vi "[ex ce] Levenberg Marquardt with independent parameter.vi"() -> ()   [LabVIEW 2021]
doc: "CE-Math example.\n\n::: CalcExpress Toolkit :::\nCopyright (c) 2000-2026 Konstantin Shifershteyn. All rights reserved."
uses:
  <vilib>/Analysis/2dsp.llb/1D Convolution (DBL).vi
  <vilib>/Analysis/NI_AALPro.lvlib
panel:
  out "error out":errorcluster
  in  "Initial Guess Coef.":cluster{"a":dbl, "b":dbl, "DC":dbl}={"a"=1.0, "b"=1.0, "DC"=0.0}
  out "Computed Coefficients":cluster{"a":dbl, "b":dbl, "DC":dbl}
  out "MSE":dbl
  in  "model description":T1={"model"="Conv( Sig , a*exp(-MesData/b)) + DC", "Parameters"=["a", "b", "DC"], "x-variable"="MesData"}
  in  "DC":dbl=4.0 caption="DC  =" format="%.1f"
  in  "Noise Amp.":dbl=2.0 caption="Noise Amplitude  =" format="%.1f"
  in  "dt, sec":dbl=0.5
  in  "a":dbl=3.0 caption="a ="
  in  "b":dbl=3.5 caption="b ="
  out "XY Graph":cluster{dbl[], dbl[]}[](graph)
  in  "Control Signal (Sig)":dbl[](array[slide])=[0.04081632653061224, 0.0510204081632653, 0.030612244897959183, 0.0510204081632653, 0.04081632653061224, 0.0510204081632653, 0.030612244897959183, 0.061224489795918366, 0.030612244897959183, 0.030612244897959183, 0.04081632653061224, 0.0510204081632653, 0.030612244897959183, 0.0510204081632653, 0.1020408163265306, 0.04081632653061224, 0.030612244897959183, 0.04081632653061224, 0.030612244897959183, 0.04081632653061224, 0.030612244897959183, 0.1020408163265306, 0.2346938775510204, 0.4387755102040816, 0.673469387755102, 0.7959183673469387, 0.9183673469387754, 0.8979591836734693, 0.8163265306122448, 0.7346938775510203, 0.6122448979591836, 0.4081632653061224, 0.24489795918367346, 0.11224489795918366, 0.061224489795918366, 0.07142857142857142, 0.07142857142857142, 0.030612244897959183, 0.0510204081632653, 0.061224489795918366, 0.07142857142857142, 0.04081632653061224, 0.030612244897959183, 0.0510204081632653, 0.0510204081632653, 0.04081632653061224, 0.030612244897959183, 0.030612244897959183, 0.061224489795918366, 0.02040816326530612, 0.030612244897959183, 0.061224489795918366, 0.030612244897959183, 0.0510204081632653, 0.030612244897959183, 0.030612244897959183, 0.02040816326530612, 0.030612244897959183, 0.04081632653061224, 0.030612244897959183, 0.04081632653061224, 0.09183673469387754, 0.2040816326530612, 0.32653061224489793, 0.4081632653061224, 0.36734693877551017, 0.25510204081632654, 0.13265306122448978, 0.061224489795918366, 0.030612244897959183, 0.030612244897959183, 0.061224489795918366, 0.0510204081632653, 0.0510204081632653, 0.0510204081632653, 0.04081632653061224, 0.04081632653061224, 0.030612244897959183, 0.02040816326530612, 0.030612244897959183, 0.030612244897959183, 0.01020408163265306, 0.0510204081632653, 0.0510204081632653, 0.030612244897959183, 0.030612244897959183, 0.030612244897959183, 0.04081632653061224, 0.0510204081632653, 0.0510204081632653, 0.030612244897959183, 0.04081632653061224, 0.030612244897959183, 0.030612244897959183, 0.030612244897959183, 0.030612244897959183, 0.04081632653061224, 0.09183673469387754, 0.04081632653061224, 0.0510204081632653, 0.04081632653061224, 0.0510204081632653, 0.04081632653061224, 0.061224489795918366, 0.04081632653061224, 0.030612244897959183, 0.030612244897959183, 0.02040816326530612, 0.04081632653061224, 0.030612244897959183, 0.02040816326530612, 0.030612244897959183, 0.08163265306122448, 0.04081632653061224, 0.04081632653061224, 0.030612244897959183, 0.030612244897959183, 0.030612244897959183, 0.030612244897959183, 0.04081632653061224, 0.061224489795918366, 0.02040816326530612, 0.030612244897959183, 0.04081632653061224, 0.04081632653061224, 0.04081632653061224, 0.04081632653061224, 0.02040816326530612, 0.04081632653061224, 0.04081632653061224, 0.04081632653061224, 0.030612244897959183, 0.04081632653061224, 0.08163265306122448, 0.04081632653061224, 0.04081632653061224, 0.04081632653061224, 0.04081632653061224, 0.04081632653061224, 0.04081632653061224, 0.0510204081632653, 0.04081632653061224, 0.04081632653061224, 0.04081632653061224, 0.04081632653061224, 0.0510204081632653, 0.04081632653061224, 0.030612244897959183, 0.030612244897959183, 0.0510204081632653] min=0.0 max=1.0 scale=0.0..1.0
  # "Measured data (MesData) conatin convolution of the\n Control Signal (Sig) and a Response Function (RF), as\n well as noise and DC component."
  # "Fitting"
  # "In order to fit Measured Data in this example, a model formula must involve Control Signal as an independent parameter (i.e. it can be evaluated in the formula but cannot be varied, like a constant).\nThis example demonstrates a technique to use independent parameters in curve fitting with the help of CalcExpress LM Fitting VI."
  # "Response function is\n   RF = a * exp(-t/b) \n, where:"
  # "Sig is an independent parameter in the model\nConv function performs a convolution"
  # "A PROCESS"
  # "Process'\nResponse\nFunction"
  # "Noise"
  # "DC"
  # "Control Signal"
  # "Measured Data"
  # "+"
  # "+"
  # "*"
  # "Convolution"
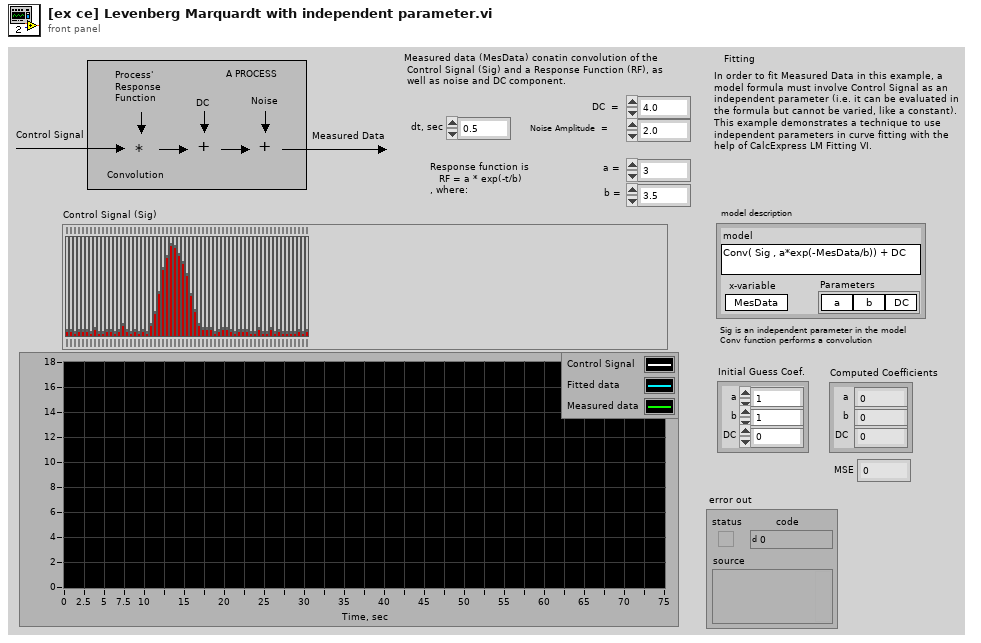
[diagram p1: front panel]
types:
  T1 = cluster{"model":string, "Parameters":string[], "x-variable":string}
  T2 = enum16{"create", "destroy", "set value", "get value"}
  T3 = typedef "VarMan Variable Context Handle.ctl" = i32
  T4 = cluster{"Best Fit Coefficients[0]":dbl, "Best Fit Coefficients[1]":dbl, "Best Fit Coefficients[2]":dbl}
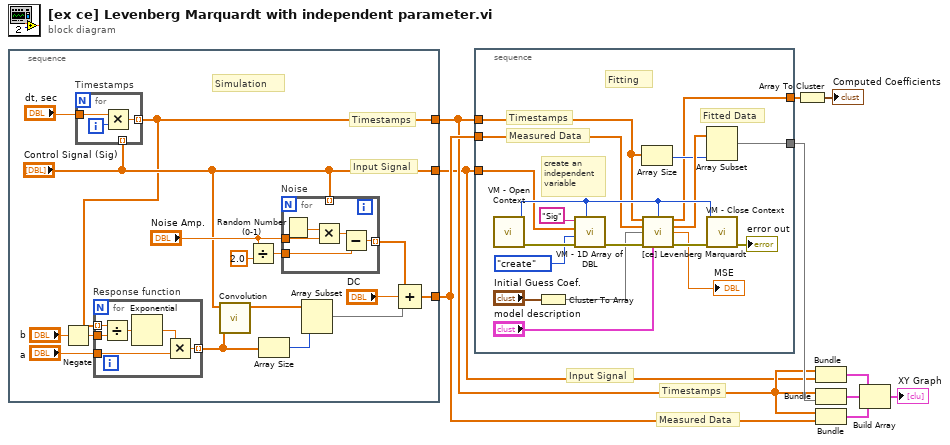
[diagram p0: block diagram]
diagram:
  # "Input Signal"
  # "Timestamps"
  # "Measured Data"
  n1 = stacked-sequence {
    tunnel: ["Control Signal (Sig)"] -> w1
    tunnel: [w14] -> w10
    tunnel: [w11] -> w3
    frame #0 {
      # "Timestamps"
      # "Input Signal"
      # "Simulation"
      n2 = Negate(x="b") -> (-x=w15:dbl)
      n3 = for "Timestamps" {
        tunnel: "dt, sec" -> [w33]
        tunnel: [w32] -> w11 mode=indexing
        tunnel: "Control Signal (Sig)" -> [_] mode=indexing
        i -> [w34]
        n4 = Multiply(x=w33, y=w34) -> (x*y=w32:dbl)
      }
      n5 = for "Response function" {
        tunnel: w11 -> [w35] mode=indexing
        tunnel: w15 -> [w39]
        tunnel: [w37] -> w16 mode=indexing
        tunnel: "a" -> [w36]
        n6 = Divide(x=w35, y=w39) -> (x/y=w40:dbl)
        n7 = Exponential(1:w40) -> (0:w38:dbl)
        n8 = Multiply(x=w38, y=w36) -> (x*y=w37:dbl)
      }
      n9 = call-poly <vilib>:"Convolution.vi"("Y"=w16, "X"="Control Signal (Sig)") -> ("X * Y"=w26:dbl[])  [unwired: 8 in, 1 out]
      n10 = Divide(x="Noise Amp.", y=2.0) -> (x/y=w21:dbl)
      n11 = Array Size(array=w16) -> (size(s)=w18:i32)
      n12 = for "Noise" {
        tunnel: "Noise Amp." -> [w29]
        tunnel: w21 -> [w28]
        tunnel: [w27] -> w17 mode=indexing
        tunnel: "Control Signal (Sig)" -> [_] mode=indexing
        n13 = Random Number (0-1)() -> (number: 0 to 1=w31:dbl)
        n14 = Multiply(x=w31, y=w29) -> (x*y=w30:dbl)
        n15 = Subtract(x=w30, y=w28) -> (x-y=w27:dbl)
      }
      n16 = Array Subset(array=w26, length=w18) -> (w19:dbl[])  [unwired: 1 in]
      n17 = Compound Arithmetic op=ADD(w17, "DC", w19) -> (w14:dbl[])
    }
  }
  n18 = stacked-sequence {
    tunnel: w3 -> [w47]
    tunnel: w1 -> [w49]
    tunnel: w10 -> [w48]
    tunnel: [w46] -> w9
    tunnel: [w45] -> w4
    frame #0 {
      # "create an\nindependent\nvariable"
      # "Fitted Data"
      # "Timestamps"
      # "Measured Data"
      # "Fitting"
      n19 = call "VM - Open Context.vi"() -> ("error out"=w58:errorcluster, "VC Handle out"=w54:T3)  [unwired: 9 in, 1 out]
      n20 = Cluster To Array(cluster="Initial Guess Coef.") -> (array=w42:dbl[])
      n21 = call "VM - 1D Array of DBL.vi"("VC Handle"=w54, "error in"=w58, "cmd"=T2."create", "value in"=w49, "name_spec"="Sig") -> ("error out"=w53:errorcluster)  [unwired: 1 in, 5 out]
      n22 = Array Size(array=w47) -> (size(s)=w51:i32)
      n23 = call "[ce] Levenberg Marquardt.vi"("X"=w47, "VC Handle"=w54, "Y"=w48, "Initial Guess Coefficients"=w42, "error in"=w53, "model description"="model description") -> ("Best Fit Coefficients"=w45:dbl[], "Best Fit"=w52:dbl[], "mse"=→"MSE":dbl, "error out"=w55:errorcluster)  [unwired: 3 in, 3 out]
      n24 = Array Subset(array=w52, length=w51) -> (w46:dbl[])  [unwired: 1 in]
      n25 = call "VM - Close Context.vi"("error in"=w55, "VC Handle"=w54) -> ("error out"=→"error out":errorcluster)  [unwired: 8 in, 1 out]
    }
  }
  n26 = Array To Cluster(array=w4) -> (cluster=→"Computed Coefficients":T4)
  n27 = Bundle(w3, "Control Signal (Sig)"=w1) -> (w2:cluster{dbl[], "Control Signal (Sig)":dbl[]})  [unwired: 1 in]
  n28 = Bundle(w3, w9) -> (w8:cluster{dbl[], dbl[]})  [unwired: 1 in]
  n29 = Bundle(w3, w10) -> (w7:cluster{dbl[], dbl[]})  [unwired: 1 in]
  n30 = Build Array(w2, w8, w7) -> (→"XY Graph":cluster{dbl[], "Control Signal (Sig)":dbl[]}[])
